vi "record.vi"() -> ()   [LabVIEW 2022 SP3]
uses:
  global_variant.vi
  <vilib>/Waveform/WDTFileIO.llb/Read Waveform from File.vi
  <vilib>/Analysis/3filter.llb/Butterworth Filter (DBL).vi
  <vilib>/Analysis/3filter.llb/Chebyshev Filter (DBL).vi
  <vilib>/Analysis/3filter.llb/Bessel Filter (DBL).vi
  <vilib>/measure/maspectr.llb/FFT Spectrum (Mag-Phase) for N Chan.vi
  <vilib>/Analysis/NI_AALBase.lvlib
  <vilib>/measure/NI_MAPro.lvlib
panel:
  out "原始波形":waveform(dbl)[](graph)
  out "是否改变波形":bool
  in  "打开波形文件":bool
  in  "加窗类型":enum16{"矩形窗", "汉宁窗", "汉明窗", "布莱克曼窗"}(ring)
  out "频谱分析":cluster{"f0":dbl, "df":dbl, "magnitude":dbl[]}[](graph)
  out "滤波结果":waveform(dbl)[](graph)
  in  "滤波器":enum16{"巴特沃斯", "切比雪夫", "贝塞尔"}(ring)
  in  "退出":bool
  # "双通道数据回放"
  # "原始波形"
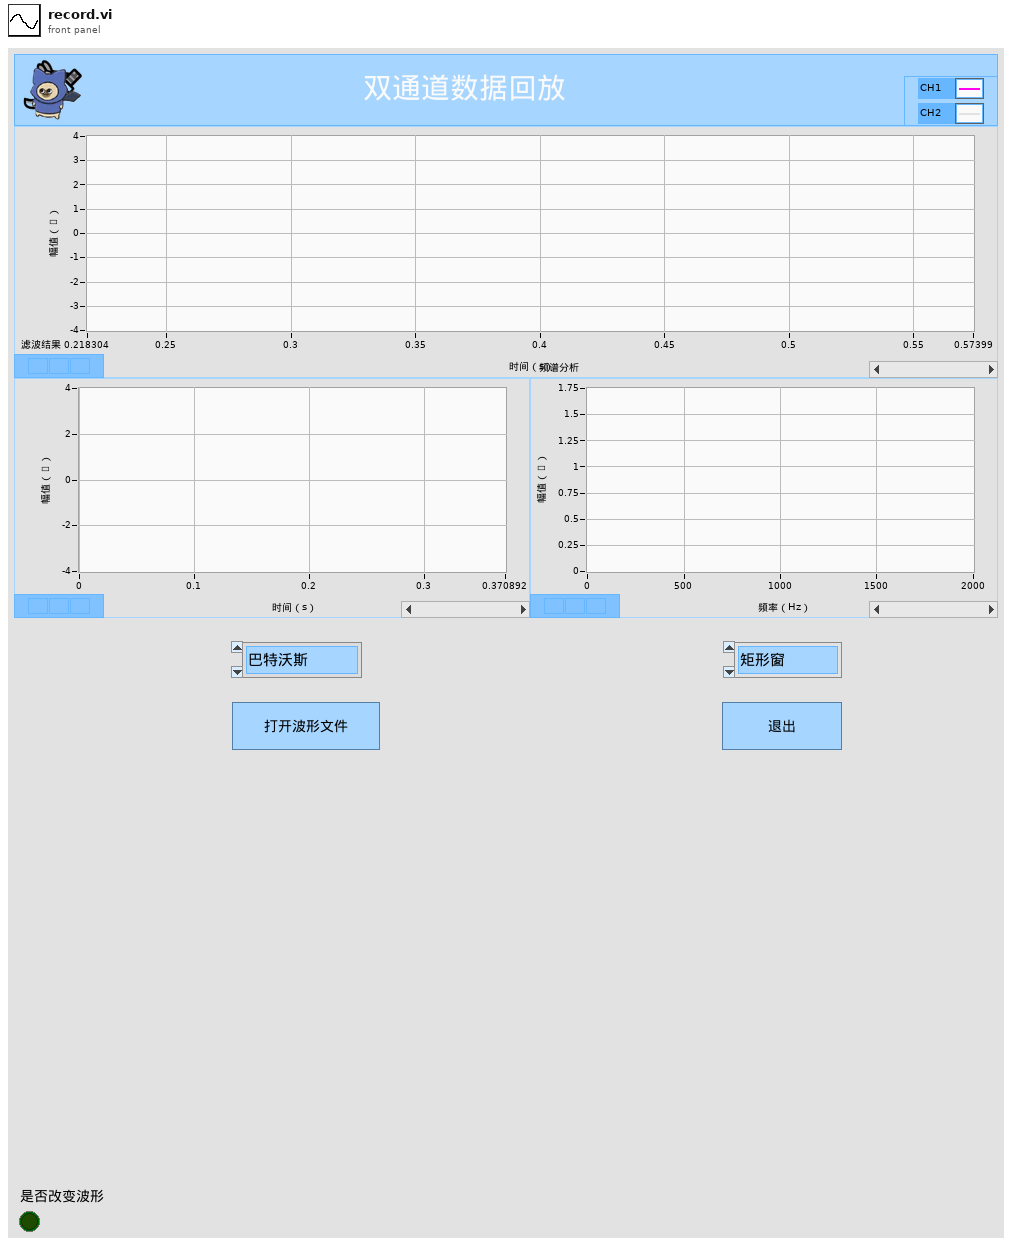
[diagram p1: front panel]
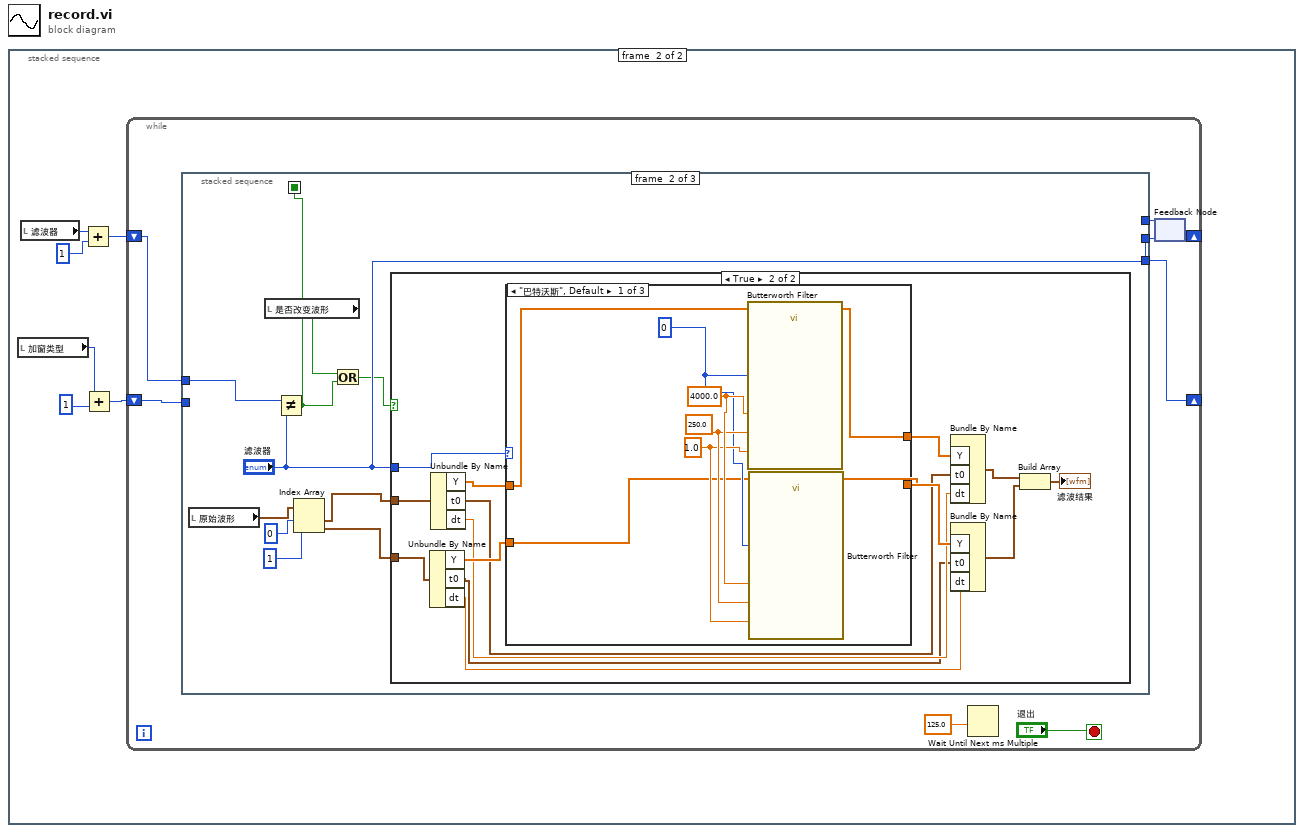
[diagram p0: block diagram]
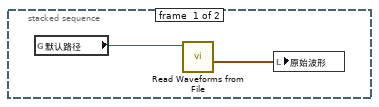
[diagram p2: hidden frame]
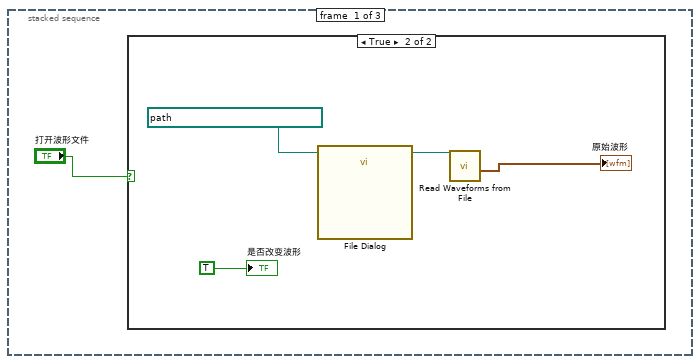
[diagram p3: hidden frame]
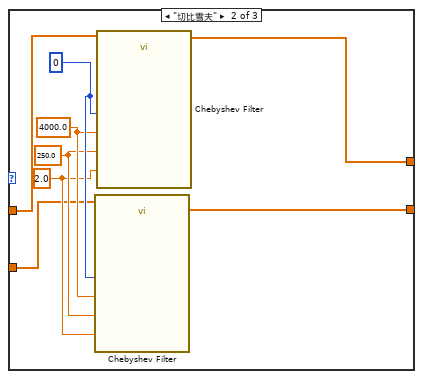
[diagram p6: hidden frame]
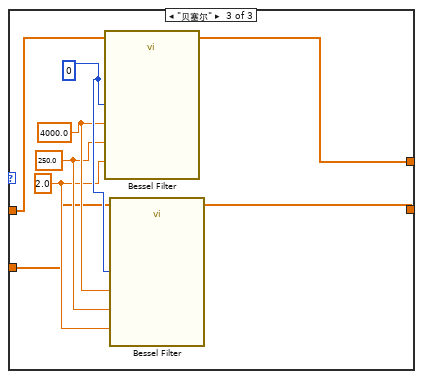
[diagram p7: hidden frame]
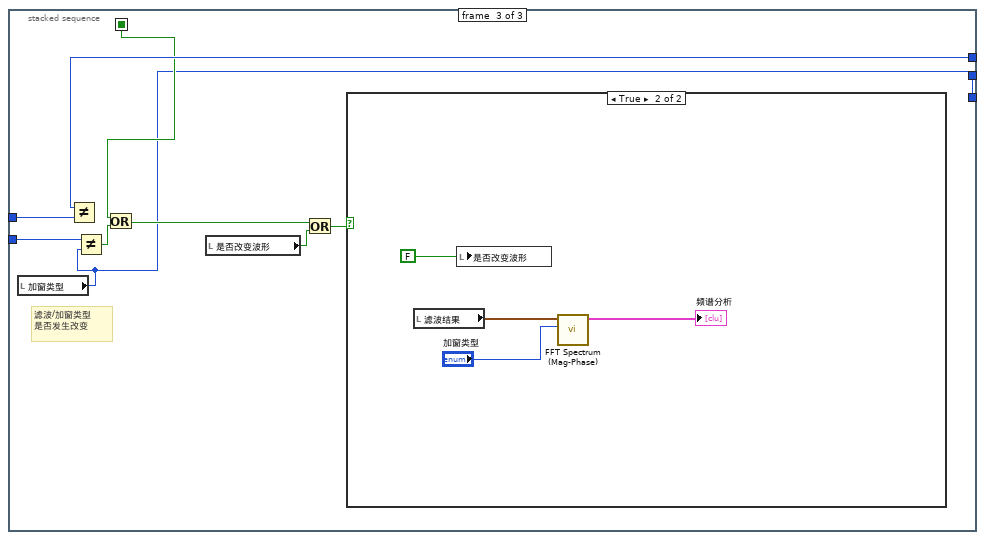
[diagram p8: hidden frame]
diagram:
  n1 = stacked-sequence {
    frame #0 {
      n2 = global read "global_variant.vi" "默认路径"() -> (w1:path)
      n3 = call-poly <vilib>:"Read Waveforms from File.vi"("file path (dialog if empty)"=w1) -> ("all waveforms in record"=w2:waveform(dbl)[])  [unwired: 5 in, 3 out]
      n4 = local write "原始波形"(w2) -> ()
    }
    frame #1 {
      n5 = local read "加窗类型"() -> (w4:enum16{"矩形窗", "汉宁窗", "汉明窗", "布莱克曼窗"})
      n6 = local read "滤波器"() -> (w8:enum16{"巴特沃斯", "切比雪夫", "贝塞尔"})
      n7 = Add(x=w8, y=1) -> (x+y=w6:i32)
      n8 = Add(x=w4, y=1) -> (x+y=w3:i32)
      n9 = while {
        shift-right: [w10] -> _
        shift-left: w6 -> [w12]
        shift-right: [w13] -> _
        shift-left: w3 -> [w9]
        stop <- "退出" stop-if-true
        n10 = Wait Until Next ms Multiple(millisecond multiple=125.0) -> ()  [unwired: 1 out]
        n11 = feedback #1() -> (w10:enum16{"巴特沃斯", "切比雪夫", "贝塞尔"})  [unwired: 1 in]
        n12 = stacked-sequence {
          seq-local: [_ w22 _] -> [_ _ w73]
          tunnel: [_ "滤波器" _] -> w11
          tunnel: [_ _ w71] -> w13
          tunnel: w12 -> [_ w30 w77]
          tunnel: w10 -> [_ _ w76]
          tunnel: w9 -> [_ _ w75]
          frame #0 {
            n13 = case shown="True" "打开波形文件" {
              frame False {
              }
              frame True {
                n14 = call "File Dialog"("start path"=path "D:/学校/LabView/DDS/saves") -> ("selected path"=w19:path)  [unwired: 11 in, 3 out]
                n15 = call-poly <vilib>:"Read Waveforms from File.vi"("file path (dialog if empty)"=w19) -> ("all waveforms in record"=→"原始波形":waveform(dbl)[])  [unwired: 5 in, 3 out]
                "是否改变波形" <- TRUE
              }
            }
          }
          frame #1 {
            n16 = local read "原始波形"() -> (w28:waveform(dbl)[])
            n17 = local read "是否改变波形"() -> (w23:bool)
            n18 = Not Equal?(x=w30, y="滤波器") -> (x != y?=w22:bool)
            n19 = Index Array(array=w28, index #1=0, index #2=1) -> (element #1=w25:waveform(dbl), element #2=w24:waveform(dbl))
            n20 = Or(x=w23, y=w22) -> (x .or. y?=w21:bool)
            n21 = case shown="True" w21 {
              tunnel: w24 -> [_ w40]
              tunnel: w25 -> [_ w41]
              tunnel: "滤波器" -> [_ w44]
              frame False {
              }
              frame True {
                n22 = Unbundle By Name(w40) -> ("Y"=w42:dbl[], "t0"=w33:timestamp, "dt"=w32:dbl)
                n23 = Unbundle By Name(w41) -> ("Y"=w43:dbl[], "t0"=w35:timestamp, "dt"=w34:dbl)
                n24 = case shown="\"巴特沃斯\", Default" w44 {
                  tunnel: [w48 w56 w63] -> w37
                  tunnel: [w47 w55 w64] -> w36
                  tunnel: w42 -> [w46 w53 w61]
                  tunnel: w43 -> [w45 w54 w62]
                  frame "巴特沃斯", Default {
                    w49 = 0
                    w51 = 250.0
                    w50 = 1.0
                    w52 = 4000.0
                    n25 = call-poly <vilib>:"Butterworth Filter.vi"("order"=w50, "filter type"=w49, "low cutoff freq: fl"=w51, "sampling freq: fs"=w52, "X"=w45) -> ("Filtered X"=w48:dbl[])  [unwired: 3 in, 1 out]
                    n26 = call-poly <vilib>:"Butterworth Filter.vi"("order"=w50, "filter type"=w49, "low cutoff freq: fl"=w51, "sampling freq: fs"=w52, "X"=w46) -> ("Filtered X"=w47:dbl[])  [unwired: 3 in, 1 out]
                  }
                  frame "切比雪夫" {
                    w60 = 0
                    w58 = 250.0
                    w57 = 2.0
                    w59 = 4000.0
                    n27 = call-poly <vilib>:"Chebyshev Filter.vi"("order"=w57, "filter type"=w60, "low cutoff freq: fl"=w58, "sampling freq: fs"=w59, "X"=w53) -> ("Filtered X"=w55:dbl[])  [unwired: 5 in, 1 out]
                    n28 = call-poly <vilib>:"Chebyshev Filter.vi"("order"=w57, "filter type"=w60, "low cutoff freq: fl"=w58, "sampling freq: fs"=w59, "X"=w54) -> ("Filtered X"=w56:dbl[])  [unwired: 5 in, 1 out]
                  }
                  frame "贝塞尔" {
                    w68 = 0
                    w66 = 250.0
                    w65 = 2.0
                    w67 = 4000.0
                    n29 = call-poly <vilib>:"Bessel Filter.vi"("order"=w65, "filter type"=w68, "low cutoff freq: fl"=w66, "sampling freq: fs"=w67, "X"=w62) -> ("Filtered X"=w63:dbl[])  [unwired: 3 in, 1 out]
                    n30 = call-poly <vilib>:"Bessel Filter.vi"("order"=w65, "filter type"=w68, "low cutoff freq: fl"=w66, "sampling freq: fs"=w67, "X"=w61) -> ("Filtered X"=w64:dbl[])  [unwired: 3 in, 1 out]
                  }
                }
                n31 = Bundle By Name("Y"=w37, "t0"=w35, "dt"=w34) -> (w39:waveform(dbl))  [unwired: 1 in]
                n32 = Bundle By Name("Y"=w36, "t0"=w33, "dt"=w32) -> (w38:waveform(dbl))  [unwired: 1 in]
                n33 = Build Array(w39, w38) -> (→"滤波结果":waveform(dbl)[])
              }
            }
          }
          frame #2 {
            # "滤波/加窗类型\n是否发生改变"
            n34 = local read "加窗类型"() -> (w71:enum16{"矩形窗", "汉宁窗", "汉明窗", "布莱克曼窗"})
            n35 = Not Equal?(x=w76, y=w77) -> ()  [unwired: 1 out]
            n36 = Not Equal?(x=w75, y=w71) -> (x != y?=w74:bool)
            n37 = Or(x=w73, y=w74) -> (x .or. y?=w72:bool)
            n38 = local read "是否改变波形"() -> (w70:bool)
            n39 = Or(x=w72, y=w70) -> (x .or. y?=w69:bool)
            n40 = case shown="True" w69 {
              frame False {
              }
              frame True {
                n41 = local read "滤波结果"() -> (w81:waveform(dbl)[])
                n42 = local write "是否改变波形"(FALSE) -> ()
                n43 = call-poly <vilib>:"FFT Spectrum (Mag-Phase).vi"("window"="加窗类型", "time signals"=w81) -> ("magnitudes"=→"频谱分析":cluster{"f0":dbl, "df":dbl, "magnitude":dbl[]}[])  [unwired: 5 in, 4 out]
              }
            }
          }
        }
        n44 = feedback-in #1(w11) -> ()
      }
    }
  }
